vi "Create StandardText Paragraph.vi"(8 "error in (no error)":errorcluster, 11 "ooWriter in":refnum<class "ooWriter.lvclass">) -> (0 "error out":errorcluster, 2 "StandardTextParagraph":refnum<k24>, 3 "ooWriter out":refnum<class "ooWriter.lvclass">)   [LabVIEW 2009, in "ooWriter.lvclass"]
uses:
  ooWriter.lvclass
  C:/Projets/LAVAG/OpenOfficeRGT/AODL/DLLs/AODL.dll
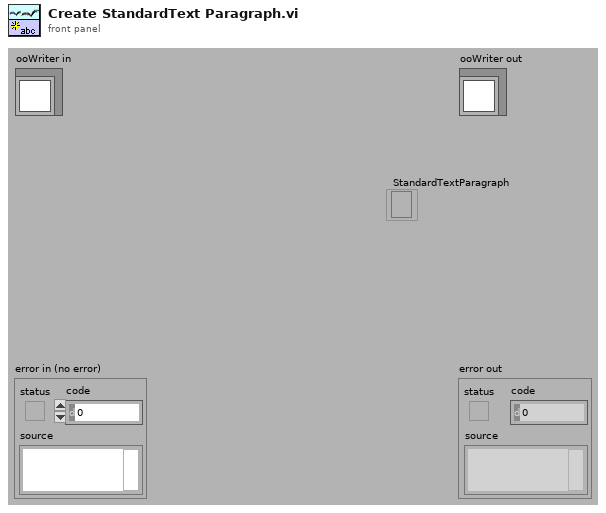
[diagram p1: front panel]
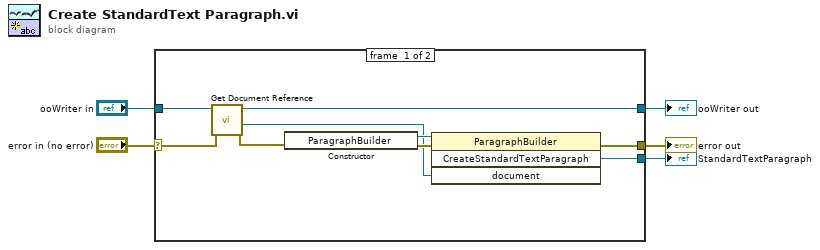
[diagram p0: block diagram]
diagram:
  n1 = case shown="No Error" "error in (no error)" {
    selector: "error in (no error)" -> [w8 w16]
    tunnel: [w6 w16] -> w4
    tunnel: [w9 w15] -> w2
    tunnel: "ooWriter in" -> [w10 w15]
    tunnel: [w12 _] -> w1
    frame #0 {
      n2 = call-dynamic "Get Document Reference.vi"("error in (no error)"=w8, "ooDocument in"=w10) -> ("error out"=w7:errorcluster, "Document"=w11:refnum<k24>, "ooDocument out"=w9:refnum<class "ooWriter.lvclass">)  [unwired: 7 in]
      n3 = constructor class="ParagraphBuilder"(error in=w7) -> (reference out=w13:refnum<k24>, error out=w14:errorcluster)  [unwired: 2 in, 1 out]
      n4 = invoke class="ParagraphBuilder" method="CreateStandardTextParagraph"(reference=w13, error in=w14, "document"=w11) -> (error out=w6:errorcluster, "CreateStandardTextParagraph"=w12:refnum<k24>)  [unwired: 1 in, 2 out]
    }
    frame #1 {
    }
  }
  "error out" <- w4
  "ooWriter out" <- w2
  "StandardTextParagraph" <- w1
